vi "AIO-Panel.vi"(7 "Set(F)":bool, 8 "error in (no error)":errorcluster, 10 "First Time(F)":bool, 11 "object in":refnum<class>) -> (0 "error out":errorcluster, 2 "Changed?":bool, 3 "object out":refnum<class>)   [LabVIEW 2021, in "AIO-Channel.lvlib" / "AIO-Configuration.lvclass"]
uses:
  AIO-Configuration.lvclass
  tdef/Data.ctl
  tdef/Direction.ctl
panel:
  out "Not Saved?":bool
  in  "Save":bool
  in  "AIOData":T1
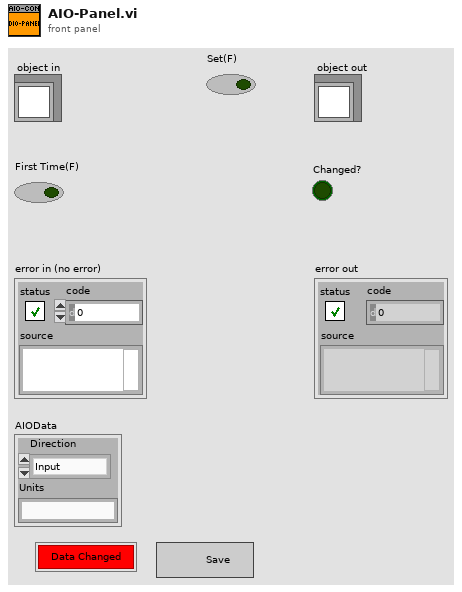
[diagram p1: front panel]
types:
  T1 = typedef "AIO-Channel.lvlib/AIO-Configuration.lvclass/Data.ctl" = cluster{"Direction":T2, "Units":string}
  T2 = typedef "AIO-Channel.lvlib/AIO-Configuration.lvclass/Direction.ctl" = enum16{"Input", "Output"}
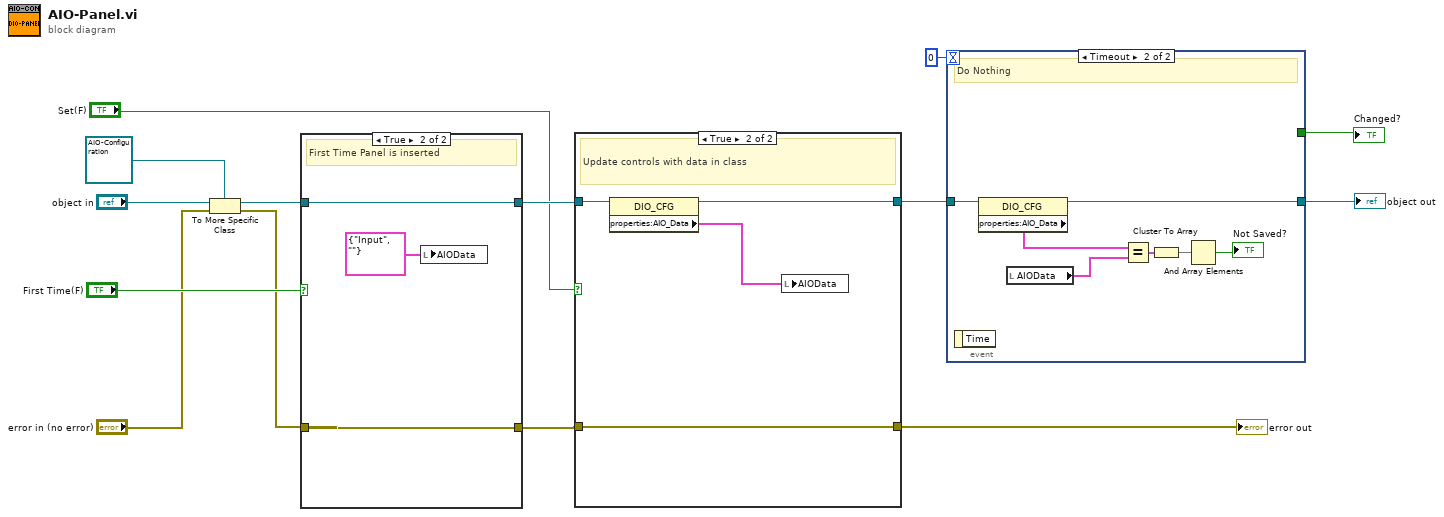
[diagram p0: block diagram]
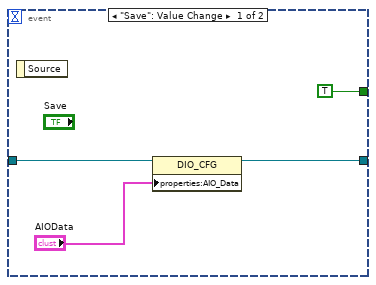
[diagram p2: hidden frame]
diagram:
  n1 = To More Specific Class(target class=refnum<class "AIO-Configuration.lvclass"> refnum ("Template-Channels.lvlib:Template_CFG"), reference="object in", error in="error in (no error)") -> (specific class reference=w8:refnum<class "AIO-Configuration.lvclass">, error out=w6:errorcluster)
  n2 = case shown="True" "First Time(F)" {
    tunnel: [w16 w19] -> w12
    tunnel: w8 -> [w16 w19]
    tunnel: [w15 w18] -> w11
    tunnel: w6 -> [w15 w18]
    frame False {
    }
    frame True {
      # "First Time Panel is inserted"
      n3 = local write "AIOData"(T1 {"Direction"=enum."Input", "Units"=""} ("TemplateData")) -> ()
    }
  }
  n4 = case shown="True" "Set(F)" {
    tunnel: [w21 w23] -> w3
    tunnel: w12 -> [w21 w25]
    tunnel: [w20 w24] -> w10
    tunnel: w11 -> [w20 w24]
    frame False {
    }
    frame True {
      # "Update controls with data in class"
      n5 = property class="DIO_CFG"(reference=w25) -> (reference out=w23:refnum<class "AIO-Configuration.lvclass">, "properties:AIO_Data"=w22:T1)  [unwired: 1 in, 1 out]
      n6 = local write "AIOData"(w22) -> ()
    }
  }
  "error out" <- w10
  n7 = event shown="[1] Timeout" {
    selector: _ -> [_ _]
    dyn-events: _ -> [_ _]
    timeout: 0 -> [_ _]
    tunnel: [w29 w35] -> w4
    tunnel: w3 -> [w28 w36]
    tunnel: [TRUE ("Changed?") _] -> w1
    event "Save": Value Change {
      n8 = event-data() -> ()  [unwired: 1 in, 1 out]
      n9 = property class="DIO_CFG"(reference=w28, "properties:AIO_Data"="AIOData") -> (reference out=w29:refnum<class "AIO-Configuration.lvclass">)  [unwired: 1 in, 1 out]
    }
    event Timeout {
      # "Do Nothing"
      n10 = event-data() -> ()  [unwired: 1 in, 1 out]
      n11 = property class="DIO_CFG"(reference=w36) -> (reference out=w35:refnum<class "AIO-Configuration.lvclass">, "properties:AIO_Data"=w34:T1)  [unwired: 1 in, 1 out]
      n12 = local read "AIOData"() -> (w33:T1)
      n13 = Equal?(x=w34, y=w33) -> (x = y?=w32:cluster{"Direction":bool, "Units":bool})
      n14 = Cluster To Array(cluster=w32) -> (array=w31:bool[])
      n15 = And Array Elements(Boolean array=w31) -> (logical AND=→"Not Saved?":bool)
    }
  }
  "object out" <- w4
  "Changed?" <- w1
